vi "from_item.vi"(8 "error in (no error)":errorcluster, 10 "item_ref":u64) -> (0 "error out":errorcluster, 3 "Value out":refnum<class "Value.lvclass">)   [LabVIEW 2020, in "toml_edit.lvlib" / "Value.lvclass"]
uses:
  Value.lvclass
  Value.lvclass/Value.ctl
  dragon_toml_64.dll
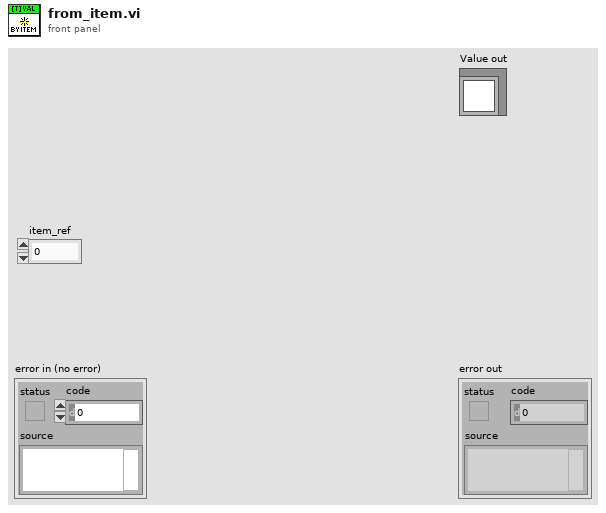
[diagram p1: front panel]
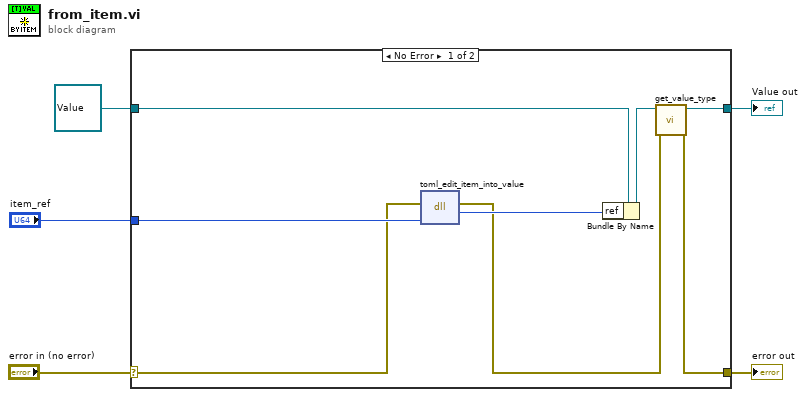
[diagram p0: block diagram]
diagram:
  n1 = case shown="No Error" "error in (no error)" {
    selector: "error in (no error)" -> [w10 w15]
    tunnel: [w6 w15] -> w4
    tunnel: [w8 w14] -> w2
    tunnel: refnum<class "Value.lvclass"> refnum ("Value in") -> [w13 w14]
    tunnel: "item_ref" -> [w12 _]
    frame No Error {
      n2 = dll-call lib="C:/projects/dragon-desktop/source/submodules/toml-edit-labview/lv_src/dragon_toml_*.dll" fn="toml_edit_item_into_value"(error in=w10, "item"=w12) -> (error out=w7:errorcluster, "value"=w11:u64)  [unwired: 3 in, 1 out]
      n3 = Bundle By Name(cluster=w13, "ref"=w11) -> (w9:refnum<class "Value.lvclass">)
      n4 = call "get_value_type.vi"("error in (no error)"=w7, "Value in"=w9) -> ("error out"=w6:errorcluster, "Value out"=w8:refnum<class "Value.lvclass">)  [unwired: 7 in, 1 out]
    }
    frame Error {
    }
  }
  "error out" <- w4
  "Value out" <- w2
